vi "PicoScope4000aGetStreamingValues.vi"(8 "error in":errorcluster, 11 "handle in":i16) -> (0 "error out":errorcluster, 1 "Trigger":cluster{bool, "triggeredAt (Total samples)":u32}, 2 "Start Index in Driver Buffer":u32, 3 "handle out":i16, 4 "Number of Samples":u32, 5 "ready":i16, 6 "Auto Stopped":bool)   [LabVIEW 2009]
doc: "This VI is used in streaming mode to get the latest values from the driver. It should be called in a loop after the oscilloscope has been set up using PicoScope4000aSettings.vi and streaming has been started by calling PicoScope4000aSetupStreaming.vi. The VI outputs the number of samples available and the start index of these samples in the array(s)."
uses:
  ps4000aWrap.dll
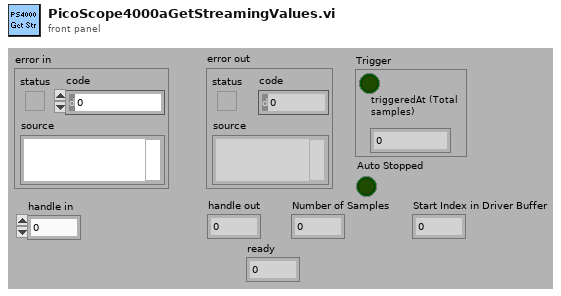
[diagram p1: front panel]
types:
  T1 = cluster{"status":bool, "code":u32, "source":string}
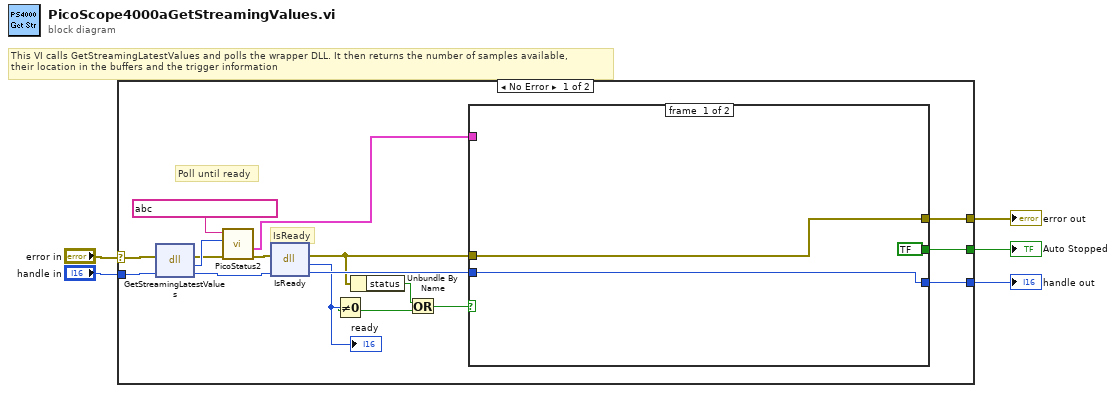
[diagram p0: block diagram]
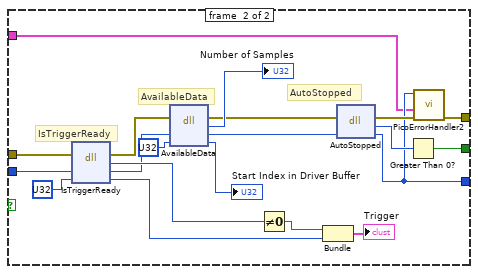
[diagram p2: hidden frame]
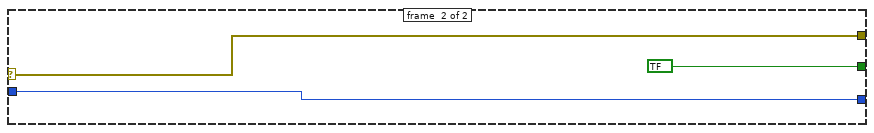
[diagram p3: hidden frame]
diagram:
  # "This VI calls GetStreamingLatestValues and polls the wrapper DLL. It then returns the number of samples available, \ntheir location in the buffers and the trigger information"
  n1 = case shown="No Error" "error in" {
    selector: "error in" -> [w17 w48]
    tunnel: [w22 w48] -> w4
    tunnel: "handle in" -> [w16 w47]
    tunnel: [w19 w47] -> w2
    tunnel: [w18 bool ?] -> w1
    frame #0 {
      # "IsReady"
      # "Poll until ready"
      n2 = dll-call lib="ps4000aWrap.dll" fn="GetStreamingLatestValues" ("PS5000.dll:_ps5000SetDataBuffer@16")(error in=w17, "handle"=w16) -> (error out=w11:errorcluster, "PICO_STATUS"=w12:u32, "handle"=w10:i16)  [unwired: 2 in, 1 out]
      n3 = call "PicoStatus2.vi"("PICO source"=string ? ("source"), "Error in"=w11, "PICO STATUS"=w12) -> ("error out"=w9:errorcluster, "PICO_STATUS out"=w6:T1)  [unwired: 5 in]
      n4 = dll-call lib="ps4000aWrap.dll" fn="IsReady" ("PS5000.dll:_ps5000SetDataBuffer@16")(error in=w9, "handle"=w10) -> (error out=w20:errorcluster, "ready"=w15:i16, "handle"=w21:i16)  [unwired: 2 in, 1 out]
      "ready" <- w15
      n5 = Not Equal To 0?(x=w15) -> (x != 0?=w13:bool)
      n6 = Unbundle By Name(w20) -> ("status"=w14:bool)
      n7 = Or(x=w14, y=w13) -> (x .or. y?=w7:bool)
      n8 = case shown="True" w7 {
        tunnel: [w24 w45] -> w22
        tunnel: w21 -> [w23 w43]
        tunnel: w20 -> [w24 w35]
        tunnel: [w23 w27] -> w19
        tunnel: [bool ? w30] -> w18
        tunnel: w6 -> [_ w26]
        frame #0 {
        }
        frame #1 {
          # "AutoStopped"
          # "AvailableData"
          # "IsTriggerReady"
          n9 = dll-call lib="ps4000aWrap.dll" fn="IsTriggerReady" ("PS5000.dll:_ps5000SetDataBuffer@16")(error in=w35, "handle"=w43, "triggeredAt"=u32 ?) -> (error out=w39:errorcluster, "triggered"=w42:i16, "handle"=w38:i16, "triggeredAt"=w28:u32)  [unwired: 2 in, 1 out]
          n10 = dll-call lib="ps4000aWrap.dll" fn="AvailableData" ("PS5000.dll:_ps5000Stop@4")(error in=w39, "handle"=w38, "startIndex"=u32 ?) -> (error out=w34:errorcluster, "numSamples"=→"Number of Samples":u32, "handle"=w32:i16, "startIndex"=→"Start Index in Driver Buffer":u32)  [unwired: 2 in, 1 out]
          n11 = Not Equal To 0?(x=w42) -> (x != 0?=w41:bool)
          n12 = Bundle(w41, "triggeredAt"=w28) -> (→"Trigger":cluster{bool, "triggeredAt":u32})  [unwired: 1 in]
          n13 = dll-call lib="ps4000aWrap.dll" fn="AutoStopped"(error in=w34, "handle"=w32) -> (error out=w33:errorcluster, "autoStopped"=w31:i16, "handle"=w27:i16)  [unwired: 2 in, 1 out]
          n14 = Greater Than 0?(x=w31) -> (x > 0?=w30:bool)
          n15 = call "PicoErrorHandler2.vi"("error in (no error)"=w33, "PICO_STATUS in"=w26, "handle In"=w27) -> ("error out"=w45:errorcluster)  [unwired: 8 in]
        }
      }
    }
    frame #1 {
    }
  }
  "error out" <- w4
  "handle out" <- w2
  "Auto Stopped" <- w1
